vi "Timer_GetAndReset.vi"(8 "Pass_Through_Time":dbl=-1.0 format="%33.4f", 11 "In Timer":T1 {"Accumulated TIme" format="%13.5p"; "StartTime" format="%13.5p"}) -> (1 "CurrentTImer":dbl, 3 "out TIMER":T1 {"Accumulated TIme" format="%13.5p"; "StartTime" format="%13.5p"})   [LabVIEW 2019, in "Trajectory_Library.lvlib"]
doc: "Synchronized call to get and reset the timer. Get the current time from the timer. If the clock is running it is derived from the current system clock the start time stored in the timer class. If the clock is not running, then return the time when it was last stopped. Also reset the timer by setting the time to 0. Make the timer startTime the current time so new requests will be relative now.\n\nInputs:\n - Timer -- The Timer data cluster\n\nOutputs:\n - Timer -- The modified Timer data cluster\n - CurrentTimer -- Current time value for this timer in seconds"
uses:
  Trajectory_Library.lvlib
  TypeDef/TIMER.ctl
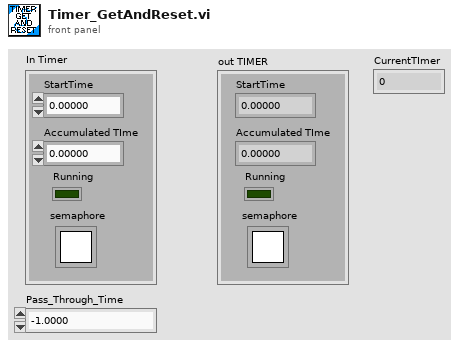
[diagram p1: front panel]
types:
  T1 = typedef "Trajectory_Library.lvlib/TIMER.ctl" = cluster{"StartTime":dbl, "Accumulated TIme":dbl, "Running":bool, "semaphore":T2}
  T2 = typedef "Semaphore RefNum" = refnum<k1>
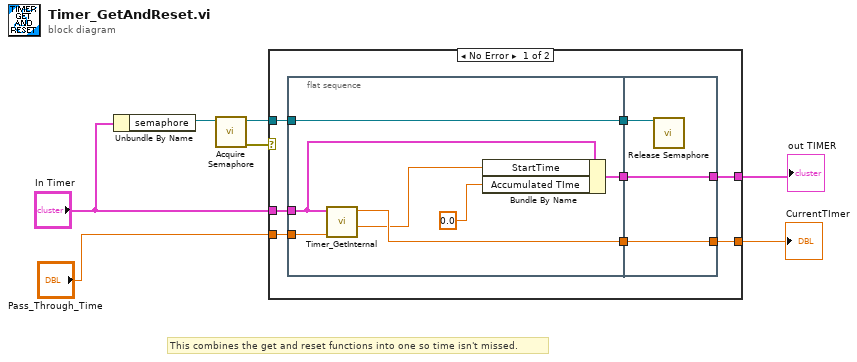
[diagram p0: block diagram]
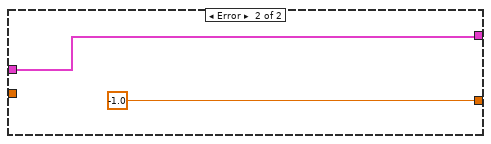
[diagram p2: hidden frame]
diagram:
  # "This combines the get and reset functions into one so time isn't missed."
  n1 = Unbundle By Name("In Timer") -> ("semaphore"=w5:T2)
  n2 = call <vilib>:"Acquire Semaphore.vi"("semaphore"=w5) -> ("error out"=w4:errorcluster, "semaphore out"=w3:T2)  [unwired: 4 in, 1 out]
  n3 = case shown="No Error" w4 {
    tunnel: [w15 -1.0 ("Accumulated TIme")] -> w7
    tunnel: "In Timer" -> [w14 w26]
    tunnel: w3 -> [w9 _]
    tunnel: [w13 w26] -> w2
    tunnel: "Pass_Through_Time" -> [w8 _]
    frame No Error {
      n4 = flat-sequence {
        tunnel: w14 -> [w21]
        tunnel: [w22] -> w12
        tunnel: [w18] -> w11
        tunnel: [w17] -> w10
        tunnel: w9 -> [w17]
        tunnel: w8 -> [w16]
        tunnel: [w24] -> w13
        tunnel: [w25] -> w15
        tunnel: w12 -> [w25]
        tunnel: w11 -> [w24]
        tunnel: w10 -> [w23]
        frame #0 {
          n5 = call "Timer_GetInternal.vi"("Pass_Through_Time"=w16, "TIMER"=w21) -> ("SystemTime"=w19:dbl, "CurrentTImer"=w22:dbl)  [unwired: 8 in]
          n6 = Bundle By Name(cluster=w21, "StartTime"=w19, "Accumulated TIme"=0.0) -> (w18:T1)
        }
        frame #1 {
          n7 = call <vilib>:"Release Semaphore.vi"("semaphore"=w23) -> ()  [unwired: 5 in, 2 out]
        }
      }
    }
    frame Error {
    }
  }
  "CurrentTImer" <- w7
  "out TIMER" <- w2
